vi "Create RDB Cluster.vi"(8 "error out":errorcluster, 11 "Channel Refs":T3[](array[typedef]) format="%.0x") -> (0 "error out":errorcluster, 3 "RDB Object":T1)   [LabVIEW 2023, in "Vires VTD System Explorer.lvlib"]
uses:
  Vires VTD System Explorer.lvlib
  <vilib>/NI VeriStand/Custom Device API/Custom Device Item Ref.ctl
  RDB Data.ctl
  RDB/RDB Player Object.ctl
  RDB/RDB Object.ctl
  RDB/RDB.lvlib
  <vilib>/NI VeriStand/Custom Device API/Custom Device API.lvlib
  Shared/Vires VTD Shared.lvlib
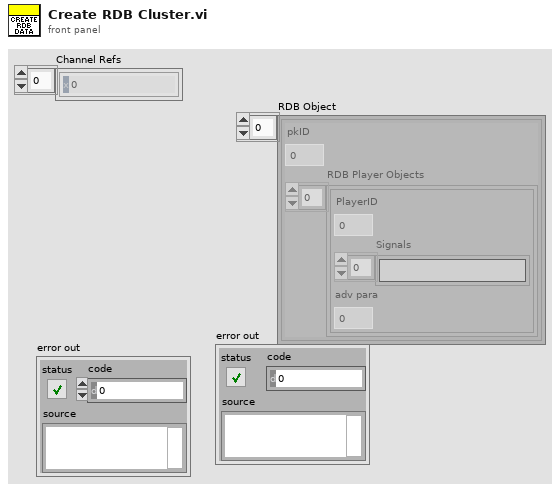
[diagram p1: front panel]
types:
  T1 = typedef "Vires VTD Shared.lvlib/RDB Data.ctl" = cluster{"pkID":i32, "RDB Player Objects":T2[]}[]
  T2 = typedef "RDB.lvlib/RDB Player Object.ctl" = cluster{"PlayerID":i32, "Signals":string[], "adv para":i32}
  T3 = typedef "Custom Device API.lvlib/Custom Device Item Ref.ctl" = u64
  T4 = typedef "RDB.lvlib/RDB Object.ctl" = cluster{"pkID":i32, "RDB Player Objects":T2[]}
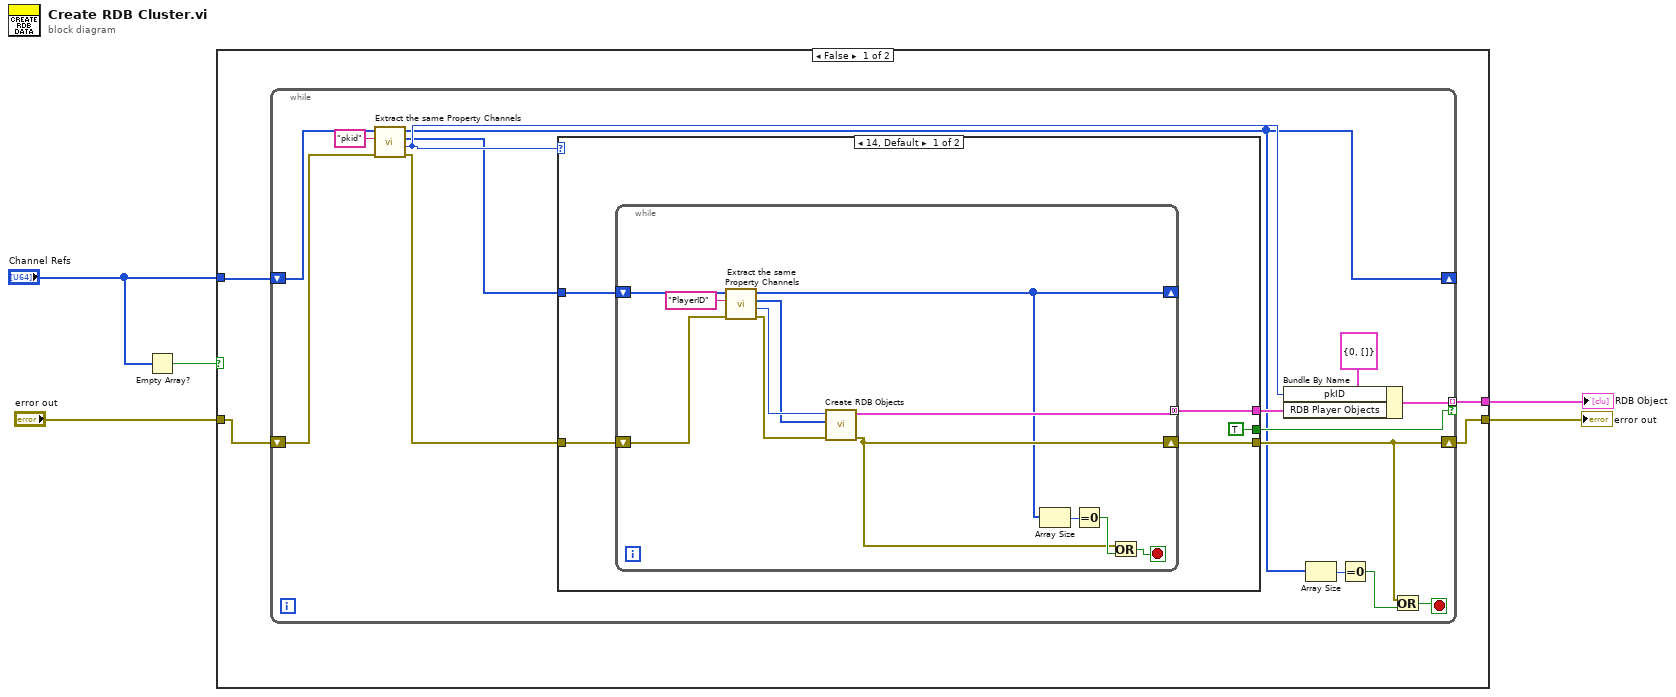
[diagram p0: block diagram]
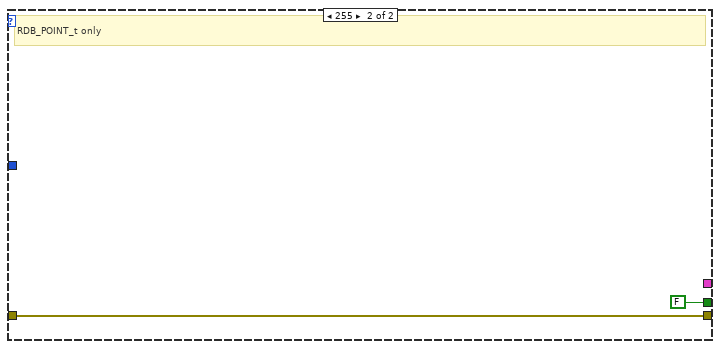
[diagram p2: hidden frame]
diagram:
  n1 = Empty Array?(array="Channel Refs") -> (empty?=w2:bool)
  n2 = case shown="False" w2 {
    tunnel: "Channel Refs" -> [w9 _]
    tunnel: "error out" -> [w8 w44]
    tunnel: [w7 w44] -> w4
    tunnel: [w6 _] -> w1
    frame False {
      n3 = while {
        shift-right: [w11] -> _
        shift-left: w9 -> [w24]
        shift-right: [w17] -> w7
        shift-left: w8 -> [w21]
        tunnel: [w16] -> w6 mode=indexing if=w13
        stop <- w18 stop-if-true
        n4 = call "Extract the same Property Channels.vi"("error in (no error)"=w21, "Property Name"="pkid", "Channel Refs in"=w24) -> ("error out"=w23:errorcluster, "Property Value"=w15:u8, "Extracted the same pkid Channel Refs"=w12:T3[], "Channel Refs Remaining"=w11:T3[])  [unwired: 5 in]
        n5 = case shown="14, Default" w15 {
          tunnel: w23 -> [w28 w43]
          tunnel: w12 -> [w29 _]
          tunnel: [w27 _] -> w22
          tunnel: [w26 w43] -> w17
          tunnel: [TRUE FALSE] -> w13
          frame 14, Default {
            n6 = while {
              shift-right: [w32] -> _
              shift-left: w29 -> [w36]
              shift-right: [w38] -> w26
              shift-left: w28 -> [w35]
              tunnel: [w37] -> w27 mode=concatenating
              stop <- w41 stop-if-true
              n7 = call "Extract the same Property Channels.vi"("error in (no error)"=w35, "Property Name"="PlayerID", "Channel Refs in"=w36) -> ("error out"=w34:errorcluster, "Property Value"=w33:u8, "Extracted the same pkid Channel Refs"=w31:T3[], "Channel Refs Remaining"=w32:T3[])  [unwired: 5 in]
              n8 = call "Create RDB Objects.vi"("error in"=w34, "Channel Refs in"=w31, "PlayerID"=w33) -> ("error out"=w38:errorcluster, "RDB OBJs"=w37:T2[])  [unwired: 7 in]
              n9 = Array Size(array=w32) -> (size(s)=w40:i32)
              n10 = Equal To 0?(x=w40) -> (x = 0?=w39:bool)
              n11 = Or(x=w38, y=w39) -> (x .or. y?=w41:bool)
            }
          }
          frame 255 {
            # "RDB_POINT_t only"
          }
        }
        n12 = Bundle By Name(cluster=T4 {"pkID"=0, "RDB Player Objects"=[]} ("RDB Object"), "pkID"=w15, "RDB Player Objects"=w22) -> (w16:T4)
        n13 = Array Size(array=w11) -> (size(s)=w19:i32)
        n14 = Equal To 0?(x=w19) -> (x = 0?=w20:bool)
        n15 = Or(x=w17, y=w20) -> (x .or. y?=w18:bool)
      }
    }
    frame True {
    }
  }
  "RDB Object" <- w1
  "error out" <- w4
